vi "Test - Text Contains.vi"(8 "error in (no error)":errorcluster, 10 "Search Text":string, 11 "Text":string) -> (0 "error out":errorcluster, 3 "Contains?":bool)   [LabVIEW 2024]
doc: "Returns TRUE when Search Text occurs in Text (case sensitive).\n\nGenerated by: Claude"
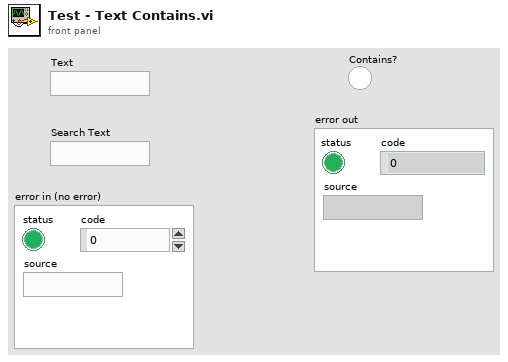
[diagram p1: front panel]
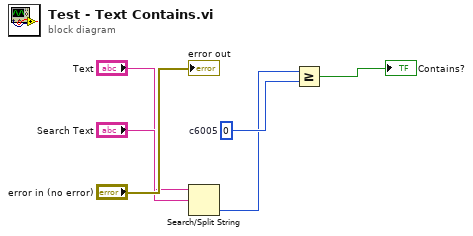
[diagram p0: block diagram]
diagram:
  w5 = 0  # c6005
  n1 = Search/Split String(string="Text", search string/char (-)="Search Text") -> (offset of match=w4:i32)  [unwired: 1 in, 2 out]
  n2 = Greater Or Equal?(x=w4, y=w5) -> (x >= y?=→"Contains?":bool)
  "error out" <- "error in (no error)"
